vi "GDSProject_GetTargetFromProjectItem.vi"(8 "error in (no error)":errorcluster, 11 "ProjectItem in":refnum<vi>) -> (0 "error out":errorcluster, 3 "TargetItem out":refnum<vi>)   [LabVIEW 2020]
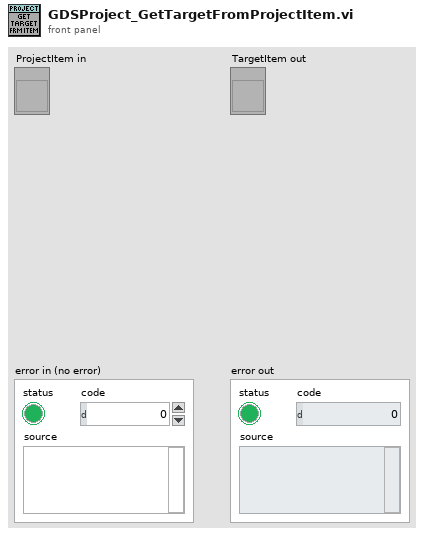
[diagram p1: front panel]
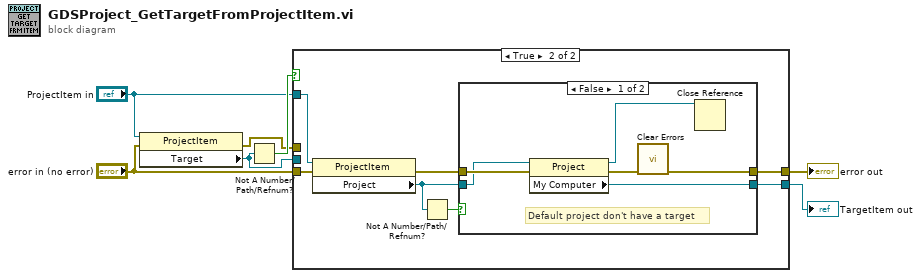
[diagram p0: block diagram]
diagram:
  n1 = property class="ProjectItem"(reference="ProjectItem in", error in="error in (no error)") -> (error out=w6:errorcluster, "Target"=w4:refnum<vi>)  [unwired: 1 out]
  n2 = Not A Number/Path/Refnum?(number/path/refnum=w4) -> (NaN/Path/Refnum?=w7:bool)
  n3 = case shown="True" w7 {
    tunnel: [w9 w15] -> w3
    tunnel: w4 -> [w9 _]
    tunnel: [w8 w16] -> w5
    tunnel: "error in (no error)" -> [_ w14]
    tunnel: w6 -> [w8 _]
    tunnel: "ProjectItem in" -> [_ w13]
    frame False {
    }
    frame True {
      n4 = property class="ProjectItem"(reference=w13, error in=w14) -> (error out=w12:errorcluster, "Project"=w11:refnum<vi>)  [unwired: 1 out]
      n5 = Not A Number/Path/Refnum?(number/path/refnum=w11) -> (NaN/Path/Refnum?=w10:bool)
      n6 = case shown="False" w10 {
        tunnel: [w17 w23] -> w16
        tunnel: [w21 _] -> w15
        tunnel: w12 -> [w20 w23]
        tunnel: w11 -> [w18 _]
        frame False {
          # "Default project don't have a target"
          n7 = property class="Project"(reference=w18, error in=w20) -> (reference out=w19:refnum<vi>, error out=w22:errorcluster, "My Computer"=w21:refnum<vi>)
          n8 = call <vilib>:"Clear Errors.vi"("error in (no error)"=w22) -> ("error out"=w17:errorcluster)  [unwired: 5 in, 1 out]
          n9 = Close Reference(reference=w19) -> ()  [unwired: 1 in, 1 out]
        }
        frame True {
        }
      }
    }
  }
  "error out" <- w5
  "TargetItem out" <- w3
